vi "ActionVIOnCompile.vi"(8 "error in (no error)":errorcluster, 11 "Device Item Ref in":T1 format="%.0x") -> (0 "error out":errorcluster)   [LabVIEW 2023, in "Vires VTD System Explorer.lvlib"]
uses:
  Vires VTD System Explorer.lvlib
  <vilib>/NI VeriStand/Custom Device API/Custom Device Item Ref.ctl
  Shared/Compiled.Settings.ctl
  RDB Data.ctl
  RDB/RDB Player Object.ctl
  Shared/Network Settings.ctl
  Shared/Protocol.ctl
  Shared/SensorInfos.ctl
  Shared/SensorInfo.ctl
  Shared/Sensor Name.ctl
  MM/MM Data.ctl
  MM/MM Objects.ctl
  MM/MM Object.ctl
  Shared/Timedloop Settings.ctl
  Shared/Constants.vi
  <vilib>/NI VeriStand/Custom Device Tools/Custom Device Utility Library/NI VeriStand - Search for Item by Name.vi
  <vilib>/NI VeriStand/Custom Device API/Get Item Property (Variant).vi
  <vilib>/NI VeriStand/Custom Device API/Set Item Property (Variant).vi
  <vilib>/NI VeriStand/Custom Device API/Custom Device API.lvlib
  <vilib>/NI VeriStand/Custom Device Tools/Custom Device Utility Library/Custom Device Utility Library.lvlib
  <vilib>/NI/NIVS Inline Async API/_Data Access System Explorer/Data Access System Explorer.lvlib
  Shared/Vires VTD Shared.lvlib
  RDB/RDB.lvlib
  MM/MM.lvlib
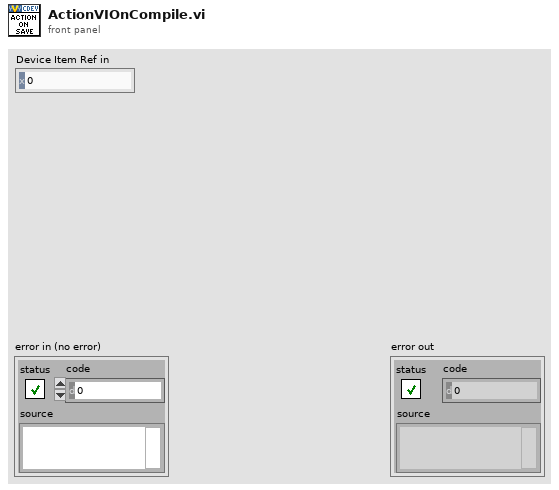
[diagram p1: front panel]
types:
  T1 = typedef "Custom Device API.lvlib/Custom Device Item Ref.ctl" = u64
  T2 = cluster{"Name":string, "Type":enum16{"Output/Write", "Input/Read", "Input/ReadWrite"}, "VS Refs":T1[]}
  T3 = enum16{"Output/Write", "Input/Read", "Input/ReadWrite"}
  T4 = typedef "Vires VTD Shared.lvlib/Compiled.Settings.ctl" = cluster{"Name":string, "RDB Data Receive ":T5, "RDB Data Sent":T5, "vclient":path, "Network Settings":T7, "SensorInfos":T9, "mmanager":path, "Scenario Paths":string[], "Custom SCP Commands":string[], "Timed Loop Settings for TaskControl":T15, "Timed Loop Settings for ModuleManager":T15}
  T5 = typedef "Vires VTD Shared.lvlib/RDB Data.ctl" = cluster{"pkID":i32, "RDB Player Objects":T6[]}[]
  T6 = typedef "RDB.lvlib/RDB Player Object.ctl" = cluster{"PlayerID":i32, "Signals":string[], "adv para":i32}
  T7 = typedef "Vires VTD Shared.lvlib/Network Settings.ctl" = cluster{"IP adress":string, "RDB":cluster{"Protocol":T8, "Tx Port":u16, "Rx Port":u16, "Buffer Size":i32, "Timeout":u16}, "SCP":cluster{"Protocol":T8, "Tx Port":u16, "Rx Port":u16, "Buffer Size":i32, "Timeout":u16}}
  T8 = typedef "Vires VTD Shared.lvlib/Protocol.ctl" = enum16{"UDP", "TCP"}
  T9 = typedef "Vires VTD Shared.lvlib/SensorInfos.ctl" = T10[]
  T10 = typedef "Vires VTD Shared.lvlib/SensorInfo.ctl" = cluster{"Sensor Name":T11, "Protocol":T8, "Network port":i32, "# Culled Objects":i32, "PlayerID":u8, "MM Data":T12}
  T11 = typedef "Vires VTD Shared.lvlib/Sensor Name.ctl" = string
  T12 = typedef "Vires VTD Shared.lvlib/MM Data.ctl" = T13[]
  T13 = typedef "MM.lvlib/MM Objects.ctl" = cluster{"pkID":i32, "MM Objects":T14[]}
  T14 = typedef "MM.lvlib/MM Object.ctl" = cluster{"Object":i32, "Signals":string[]}
  T15 = typedef "Vires VTD Shared.lvlib/Timedloop Settings.ctl" = cluster{"Period(ms)":i64, "Priority":i32, "Processor":i32}
  T16 = typedef "Custom Device API.lvlib/Custom Device Item Info.ctl" = cluster{"Name":string, "Is Channel":bool, "GUID":string, "Is Waveform":bool}
  T17 = cluster{"Name":string, "Type":enum16{"Output/Write", "Input/Read", "Input/ReadWrite"}, "VS Refs":T1[]}[]
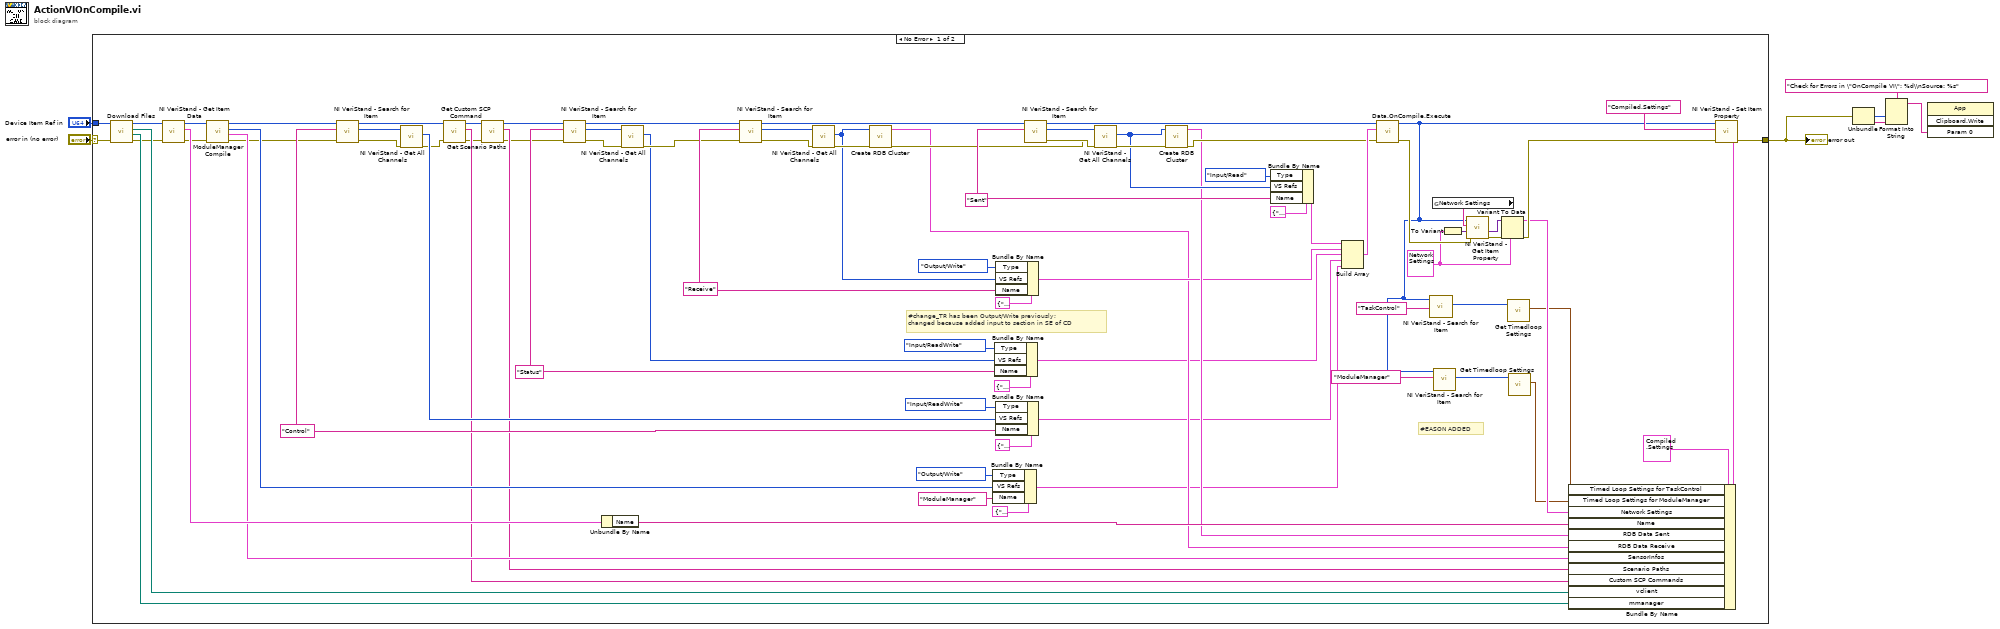
[diagram p0: block diagram]
diagram:
  n1 = case shown="No Error" "error in (no error)" {
    selector: "error in (no error)" -> [w61 w92]
    tunnel: [w63 w92] -> w3
    tunnel: "Device Item Ref in" -> [w62 _]
    frame No Error {
      w27 = "Control" ("Item Name")
      w48 = "Status" ("Item Name")
      w37 = T7 {"IP adress"="127.0.0.1", "RDB"={"Protocol"=enum."UDP", "Tx Port"=48190, "Rx Port"=8192, "Buffer Size"=48190, "Timeout"=10}, "SCP"={"Protocol"=enum."UDP", "Tx Port"=48190, "Rx Port"=8192, "Buffer Size"=48190, "Timeout"=10}} ("UDP Settings")
      w86 = "Sent" ("Item Name")
      w87 = "Receive" ("Item Name")
      # "#EASON ADDED"
      # "#change_TR has been Output/Write previously;\nchanged because added input to section in SE of CD"
      n2 = call "Download Files.vi"("error in (no error)"=w61, "Item Ref in"=w62) -> ("error out"=w17:errorcluster, "mmanager"=w38:path, "vclient"=w40:path, "Device Ref out"=w60:T1)  [unwired: 6 in]
      n3 = call <vilib>:"NI VeriStand - Get Item Data.vi"("error in (no error)"=w17, "Item Ref in"=w60) -> ("error out"=w45:errorcluster, "Item Info"=w89:T16, "Item Ref out"=w46:T1)  [unwired: 6 in, 1 out]
      n4 = call "ModuleManager Compile.vi"("error in"=w45, "Section Ref in"=w46) -> ("error out"=w25:errorcluster, "SensorInfos"=w39:T9, "Channel Refs"=w42:T1[], "Section Ref out"=w28:T1)  [unwired: 6 in]
      n5 = call-poly <vilib>:"NI VeriStand - Search for Item.vi"("error in"=w25, "Item Name"=w27, "Section Ref in"=w28) -> ("error out"=w30:errorcluster, "Item Ref"=w29:T1, "Section Ref out"=w21:T1)  [unwired: 5 in, 1 out]
      n6 = call <vilib>:"NI VeriStand - Get All Channels.vi"("error in"=w30, "Section Ref in"=w29) -> ("error out"=w24:errorcluster, "Channel Refs"=w26:T1[])  [unwired: 6 in, 2 out]
      n7 = call "Get Custom SCP Command.vi"("error in (no error)"=w24, "Section Ref in"=w21) -> ("error out"=w15:errorcluster, "Custom SCP Commands (str)"=w19:string[], "Section Ref out"=w20:T1)  [unwired: 7 in]
      n8 = call "Get Scenario Paths.vi"("error in (no error)"=w15, "Section Ref in"=w20) -> ("error out"=w16:errorcluster, "Scenario Paths (str)"=w18:string[], "Section Ref out"=w23:T1)  [unwired: 6 in, 1 out]
      n9 = call-poly <vilib>:"NI VeriStand - Search for Item.vi"("error in"=w16, "Item Name"=w48, "Section Ref in"=w23) -> ("error out"=w54:errorcluster, "Item Ref"=w55:T1, "Section Ref out"=w53:T1)  [unwired: 5 in, 1 out]
      n10 = Unbundle By Name(w89) -> ("Name"=w88:string)
      n11 = call <vilib>:"NI VeriStand - Get All Channels.vi"("error in"=w54, "Section Ref in"=w55) -> ("error out"=w52:errorcluster, "Channel Refs"=w49:T1[])  [unwired: 6 in, 2 out]
      n12 = call-poly <vilib>:"NI VeriStand - Search for Item.vi"("error in"=w52, "Item Name"=w87, "Section Ref in"=w53) -> ("error out"=w76:errorcluster, "Item Ref"=w75:T1, "Section Ref out"=w78:T1)  [unwired: 5 in, 1 out]
      n13 = call <vilib>:"NI VeriStand - Get All Channels.vi"("error in"=w76, "Section Ref in"=w75) -> ("error out"=w72:errorcluster, "Channel Refs"=w71:T1[])  [unwired: 6 in, 2 out]
      n14 = call "Create RDB Cluster.vi"("error out"=w72, "Channel Refs"=w71) -> ("error out"=w70:errorcluster, "RDB Object"=w64:T5)  [unwired: 8 in]
      n15 = Bundle By Name(cluster=T2 {"Name"="", "Type"=enum."Output/Write", "VS Refs"=[]} ("Group"), "Type"=T3."Output/Write", "VS Refs"=w42, "Name"="ModuleManager") -> (w34:T2)
      n16 = Bundle By Name(cluster=T2 {"Name"="", "Type"=enum."Output/Write", "VS Refs"=[]} ("Group"), "Type"=T3."Input/ReadWrite", "VS Refs"=w49, "Name"=w48) -> (w47:T2)
      n17 = Bundle By Name(cluster=T2 {"Name"="", "Type"=enum."Output/Write", "VS Refs"=[]} ("Group"), "Type"=T3."Output/Write", "VS Refs"=w71, "Name"=w87) -> (w65:T2)
      n18 = Bundle By Name(cluster=T2 {"Name"="", "Type"=enum."Output/Write", "VS Refs"=[]} ("Group"), "Type"=T3."Input/ReadWrite", "VS Refs"=w26, "Name"=w27) -> (w31:T2)
      n19 = call-poly <vilib>:"NI VeriStand - Search for Item.vi"("error in"=w70, "Item Name"=w86, "Section Ref in"=w78) -> ("error out"=w74:errorcluster, "Item Ref"=w73:T1, "Section Ref out"=w79:T1)  [unwired: 5 in, 1 out]
      n20 = call <vilib>:"NI VeriStand - Get All Channels.vi"("error in"=w74, "Section Ref in"=w73) -> ("error out"=w69:errorcluster, "Channel Refs"=w68:T1[])  [unwired: 6 in, 2 out]
      n21 = call "Create RDB Cluster.vi"("error out"=w69, "Channel Refs"=w68) -> ("error out"=w67:errorcluster, "RDB Object"=w66:T5)  [unwired: 8 in]
      n22 = Bundle By Name(cluster=T2 {"Name"="", "Type"=enum."Output/Write", "VS Refs"=[]} ("Group"), "Type"=T3."Input/Read", "VS Refs"=w68, "Name"=w86) -> (w84:T2)
      n23 = Build Array(w84, w65, w47, w31, w34) -> (w82:T17)
      n24 = call <vilib>:"Data.OnCompile.Execute.vi"("error in"=w67, "VS Ref Groups"=w82, "Custom Device Ref"=w79) -> ("error out"=w56:errorcluster, "Custom Device Ref"=w14:T1)  [unwired: 7 in]
      n25 = call-poly <vilib>:"NI VeriStand - Search for Item.vi"("Item Name"="TaskControl", "Section Ref in"=w14) -> ("Item Ref"=w13:T1)  [unwired: 6 in, 3 out]
      n26 = global read "Constants.vi" "Network Settings"() -> (w59:string)
      n27 = call-poly <vilib>:"NI VeriStand - Search for Item.vi"("Item Name"="ModuleManager", "Section Ref in"=w14) -> ("Item Ref"=w12:T1)  [unwired: 6 in, 3 out]
      n28 = To Variant(anything=w37) -> (Variant=w36:variant)
      n29 = call-poly <vilib>:"NI VeriStand - Get Item Property.vi"("error in (no error)"=w56, "Default Value"=w36, "Property Name"=w59, "Item Ref in"=w14) -> ("error out"=w58:errorcluster, "Value"=w57:variant)  [unwired: 4 in, 2 out]
      n30 = Variant To Data(error in=w58, type=w37, Variant=w57) -> (data=w22:T7, error out=w35:errorcluster)
      n31 = call "Get Timedloop Settings.vi"("Item Ref in"=w13) -> ("Timed Loop Settings"=w8:T15)  [unwired: 8 in, 2 out]
      n32 = call "Get Timedloop Settings.vi"("Item Ref in"=w12) -> ("Timed Loop Settings"=w9:T15)  [unwired: 8 in, 2 out]
      n33 = Bundle By Name(cluster=T4 {"Name"="", "RDB Data Receive "=[], "RDB Data Sent"=[], "vclient"=path "", "Network Settings"={"IP adress"="127.0.0.1", "RDB"={"Protocol"=enum."UDP", "Tx Port"=48190, "Rx Port"=10, "Buffer Size"=204800, "Timeout"=10}, "SCP"={"Protocol"=enum."TCP", "Tx Port"=48191, "Rx Port"=48191, "Buffer Size"=204800, "Timeout"=10}}, "SensorInfos"=[], "mmanager"=path "", "Scenario Paths"=[], "Custom SCP Commands"=[], "Timed Loop Settings for TaskControl"={"Period(ms)"=2, "Priority"=100, "Processor"=-2}, "Timed Loop Settings for ModuleManager"={"Period(ms)"=2, "Priority"=100, "Processor"=-2}} ("Compiled.Settings"), "Timed Loop Settings for TaskControl"=w8, "Timed Loop Settings for ModuleManager"=w9, "Network Settings"=w22, "Name"=w88, "RDB Data Sent"=w66, "RDB Data Receive"=w64, "SensorInfos"=w39, "Scenario Paths"=w18, "Custom SCP Commands"=w19, "vclient"=w40, "mmanager"=w38) -> (w90:T4)
      n34 = call-poly <vilib>:"NI VeriStand - Set Item Property.vi"("error in (no error)"=w35, "Value"=w90, "Property Name"="Compiled.Settings", "Item Ref in"=w14) -> ("error out"=w63:errorcluster)  [unwired: 5 in, 2 out]
    }
    frame Error {
    }
  }
  "error out" <- w3
  n35 = Unbundle(w3) -> ("code"=w4:i32, "source"=w5:string)  [unwired: 1 out]
  n36 = Format Into String(format string="Check for Errors in \"OnCompile VI\": %d\\nSource: %s", w4, w5) -> (resulting string=w2:string)  [unwired: 2 in, 1 out]
  n37 = invoke class="App" method="Clipboard.Write"("Param 0"=w2) -> ()  [unwired: 3 in, 4 out]
